vi "test_Set Turn Table Scan Speed.vi"(8 "error in (no error)":errorcluster, 11 "TestCase in":refnum<class "EM1000 Turn Table.lvclass">) -> (0 "error out":errorcluster, 3 "TestCase out":refnum<class "EM1000 Turn Table.lvclass">)   [LabVIEW 2020, in "EM1000 Turn Table.lvclass"]
uses:
  EM1000 Turn Table.lvclass
  EM1000 Turn Table.lvclass/EM1000 Turn Table.ctl
  AUDIX EM1000.lvclass/AUDIX EM1000.ctl
  AUDIX EM1000.lvclass
  <vilib>/addons/_JKI Toolkits/VI Tester/TestCase.llb/TestCase.lvclass
  C:/Program Files (x86)/National Instruments/LabVIEW 2020/vi.lib/addons/_JKI Toolkits/VI Tester/TestCase.llb/TestCase.lvclass
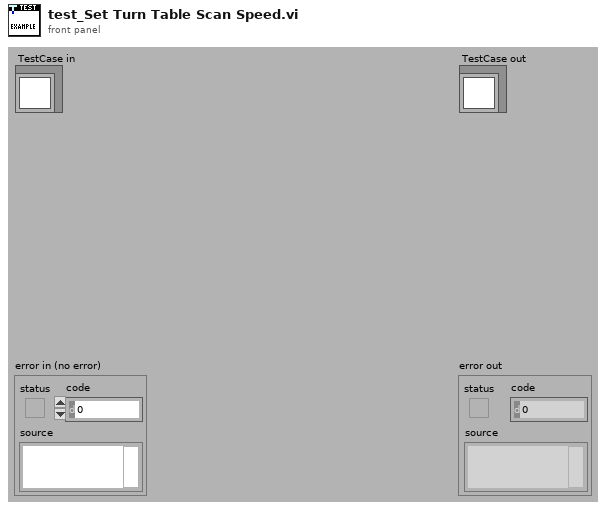
[diagram p1: front panel]
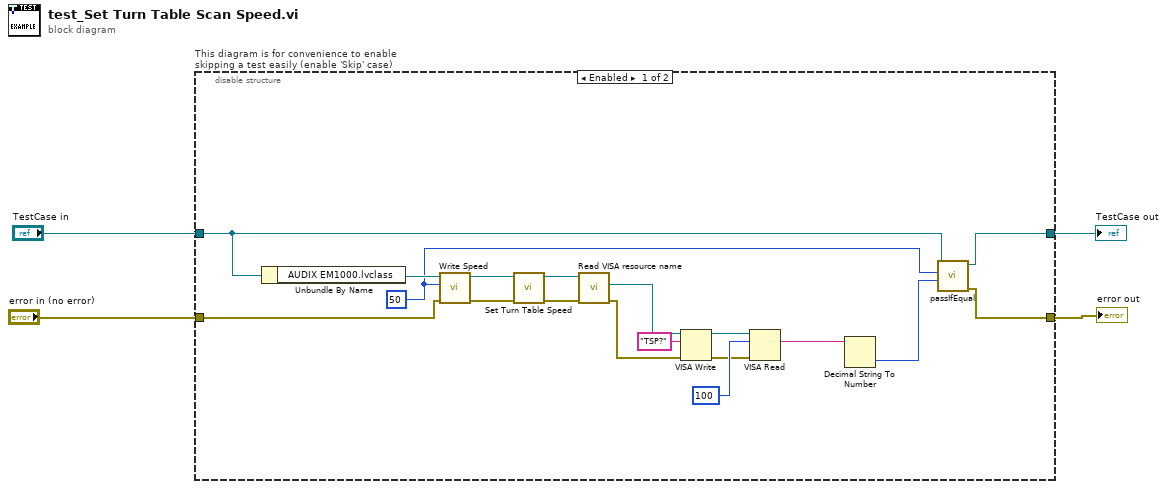
[diagram p0: block diagram]
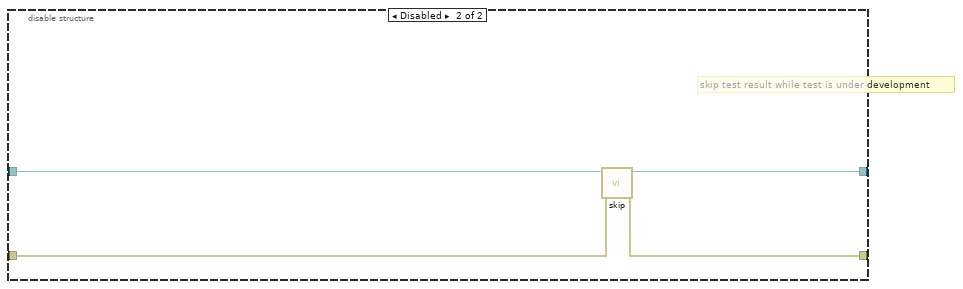
[diagram p2: hidden frame]
diagram:
  n1 = disable-structure "This diagram is for convenience to enable skipping a test easily (enable 'Skip' case)" shown="Enabled" {
    disable-tunnel: "TestCase in" -> [w22 w26]
    disable-tunnel: [w8 w24] -> w1
    disable-tunnel: [w7 w25] -> w3
    disable-tunnel: "error in (no error)" -> [w20 w23]
    frame Enabled {
      w9 = 50 ("Speed")
      n2 = Unbundle By Name(w22) -> ("AUDIX EM1000.lvclass"=w21:refnum<class "AUDIX EM1000.lvclass">)
      n3 = call "Write Speed.vi"("error in (no error)"=w20, "Speed"=w9, "AUDIX EM1000 in"=w21) -> ("error out"=w18:errorcluster, "AUDIX EM1000 out"=w19:refnum<class "AUDIX EM1000.lvclass">)  [unwired: 7 in]
      n4 = call-dynamic "Set Turn Table Speed.vi"("error in (no error)"=w18, "AUDIX EM1000 in"=w19) -> ("error out"=w16:errorcluster, "AUDIX EM1000 out"=w17:refnum<class "AUDIX EM1000.lvclass">)  [unwired: 8 in]
      n5 = call "Read VISA resource name.vi"("error in (no error)"=w16, "AUDIX EM1000 in"=w17) -> ("error out"=w13:errorcluster, "VISA resource name"=w15:refnum<visa-resource-name>)  [unwired: 7 in, 1 out]
      n6 = VISA Write(VISA resource name=w15, write buffer="TSP?", error in (no error)=w13) -> (VISA resource name out=w12:refnum<visa-resource-name>, error out=w10:errorcluster)  [unwired: 1 out]
      n7 = VISA Read(VISA resource name=w12, byte count=u32 100, error in (no error)=w10) -> (read buffer=w6:string)  [unwired: 3 out]
      n8 = Decimal String To Number(string=w6) -> (number=w5:i32)  [unwired: 2 in, 1 out]
      n9 = call-dynamic "passIfEqual.vi"("y"=w5, "x"=w9, "TestCase in"=w22) -> ("error out"=w7:errorcluster, "TestCase out"=w8:refnum<class "EM1000 Turn Table.lvclass">)  [unwired: 7 in]
    }
    frame Disabled {
      # "skip test result while test is under development"
      n10 = call <vilib>:"skip.vi"("error in (no error)"=w23, "TestCase in"=w26) -> ("error out"=w25:errorcluster, "TestCase out"=w24:refnum<class "EM1000 Turn Table.lvclass">)  [unwired: 8 in]
    }
  }
  "error out" <- w3
  "TestCase out" <- w1
